vi "onDisconnection.vi"(8 "error in (no error)":errorcluster, 11 "Connection":refnum<class "Connection.lvclass">) -> (0 "error out":errorcluster, 3 "No connection":refnum<class "Connection.lvclass">)   [LabVIEW 2013, in "Connection_GOSPL.lvlib" / "Connection.lvclass"]
uses:
  Connection.lvclass
  Connection.lvclass/Connection.ctl
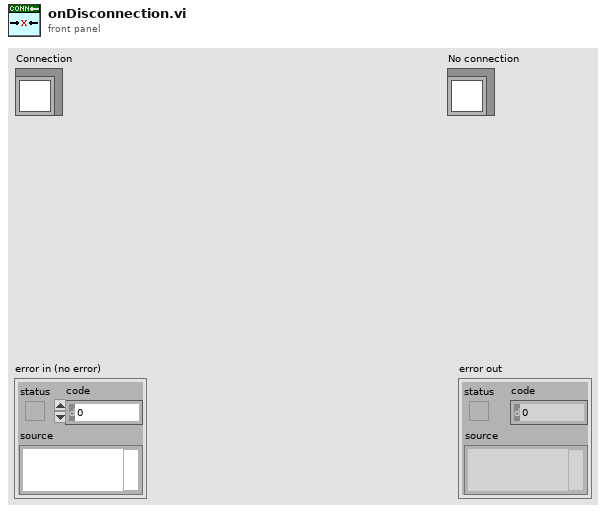
[diagram p1: front panel]
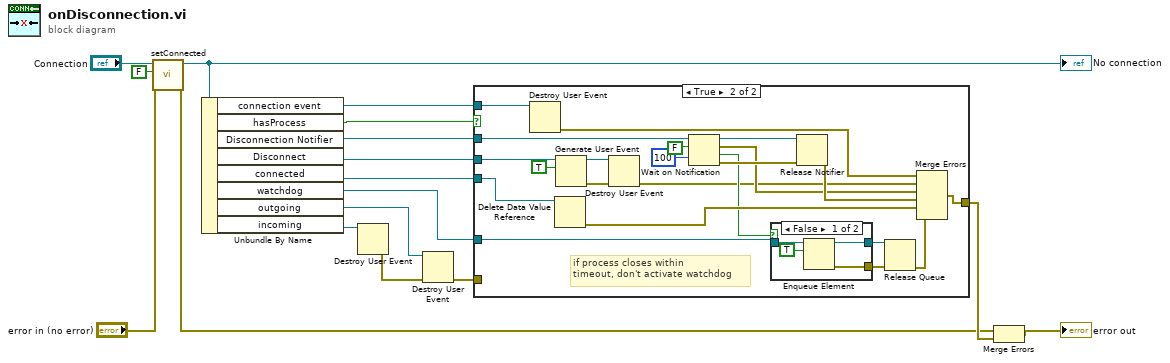
[diagram p0: block diagram]
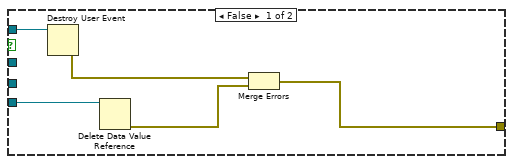
[diagram p2: hidden frame]
diagram:
  n1 = call "setConnected.vi"("error in (no error)"="error in (no error)", "connected"=FALSE, "Connection in"="Connection") -> ("error out"=w6:errorcluster, "Connection out"=w8:refnum<class "Connection.lvclass">)  [unwired: 7 in]
  "No connection" <- w8
  n2 = Unbundle By Name(w8) -> ("connection event"=w5:refnum<user-event>, "hasProcess"=w13:bool, "Disconnection Notifier"=w16:refnum<notifier>, "Disconnect"=w17:refnum<user-event>, "connected"=w12:refnum<data-value>, "watchdog"=w11:refnum<queue>, "outgoing"=w4:refnum<user-event>, "incoming"=w3:refnum<user-event>)
  n3 = Destroy User Event(user event=w3) -> (error out=w1:errorcluster)  [unwired: 1 in]
  n4 = Destroy User Event(user event=w4, error in=w1) -> (error out=w2:errorcluster)
  n5 = case shown="True" w13 {
    tunnel: w17 -> [_ w44]
    tunnel: w16 -> [_ w43]
    tunnel: [w18 w37] -> w15
    tunnel: w12 -> [w22 w36]
    tunnel: w11 -> [_ w32]
    tunnel: w5 -> [w21 w27]
    tunnel: w2 -> [_ _]
    frame False {
      n6 = Destroy User Event(user event=w21) -> (error out=w20:errorcluster)  [unwired: 1 in]
      n7 = Delete Data Value Reference(data value reference=w22) -> (error out=w19:errorcluster)  [unwired: 1 in, 1 out]
      n8 = Merge Errors(w20, w19) -> (w18:errorcluster)
    }
    frame True {
      # "if process closes within\ntimeout, don't activate watchdog"
      n9 = Destroy User Event(user event=w27) -> (error out=w26:errorcluster)  [unwired: 1 in]
      n10 = Delete Data Value Reference(data value reference=w36) -> (error out=w35:errorcluster)  [unwired: 1 in, 1 out]
      n11 = Generate User Event(user event=w44, event data cluster=TRUE ("event data")) -> (user event out=w24:refnum<user-event>, error out=w25:errorcluster)  [unwired: 2 in]
      n12 = Destroy User Event(user event=w24, error in=w25) -> (error out=w23:errorcluster)
      n13 = Wait on Notification(notifier=w43, ignore previous (F)=FALSE, timeout in ms (-1)=100) -> (notifier out=w39:refnum<notifier>, notification=w33:errorcluster, timed out?=w28:bool, error out=w34:errorcluster)  [unwired: 1 in]
      n14 = case shown="False" w28 {
        tunnel: w32 -> [w48 w49]
        tunnel: [w47 w49] -> w31
        tunnel: [w45 _] -> w30
        frame False {
          n15 = Enqueue Element(queue=w48, element=TRUE) -> (queue out=w47:refnum<queue>, error out=w45:errorcluster)  [unwired: 2 in, 1 out]
        }
        frame True {
        }
      }
      n16 = Release Notifier(notifier=w39, error in (no error)=w34) -> (error out=w38:errorcluster)  [unwired: 1 in, 2 out]
      n17 = Release Queue(queue=w31, error in (no error)=w30) -> (error out=w29:errorcluster)  [unwired: 1 in, 2 out]
      n18 = Merge Errors(w26, w23, w33, w38, w35, w29) -> (w37:errorcluster)
    }
  }
  n19 = Merge Errors(w6, w15) -> (→"error out":errorcluster)
